vi "Read Boolean.vi"(8 "error in":errorcluster, 9 "RegisterOffset":u32, 10 "register name":string, 11 "session in":u32) -> (0 "error out":errorcluster, 2 "value out":bool, 3 "session out":u32)   [LabVIEW 2020, in "FPGA Register IO.lvlib"]
uses:
  FPGA Register IO.lvlib
  NiFpga.dll
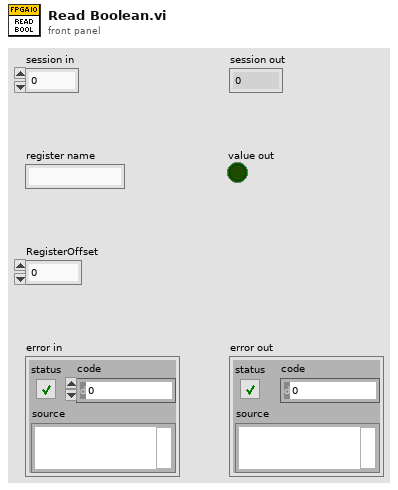
[diagram p1: front panel]
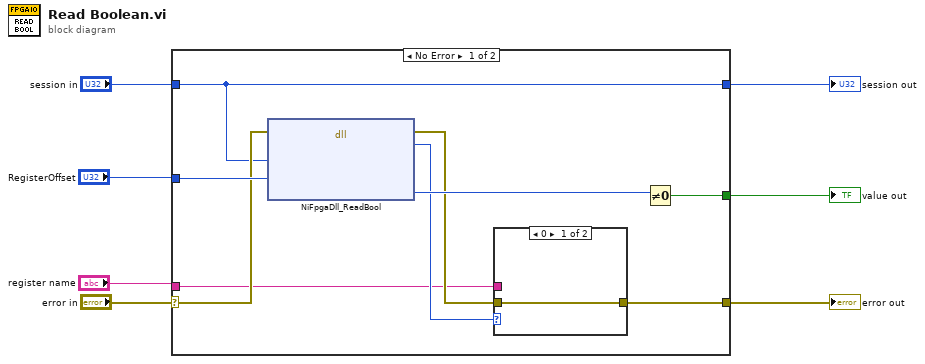
[diagram p0: block diagram]
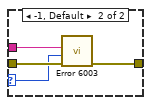
[diagram p2: hidden frame]
diagram:
  n1 = case shown="No Error" "error in" {
    selector: "error in" -> [w15 w23]
    tunnel: "session in" -> [w14 w22]
    tunnel: [w9 w23] -> w7
    tunnel: [w13 _] -> w5
    tunnel: "RegisterOffset" -> [w16 _]
    tunnel: [w14 w22] -> w6
    tunnel: "register name" -> [w8 _]
    frame No Error {
      n2 = dll-call lib="NiFpga.*" fn="NiFpgaDll_ReadBool"(error in=w15, "session"=w14, "offset"=w16) -> (error out=w10:errorcluster, "status"=w11:i32, "value"=w12:u8)  [unwired: 5 in, 1 out]
      n3 = case shown="0" w11 {
        selector: w11 -> [_ w18]
        tunnel: w10 -> [w17 w21]
        tunnel: [w17 w20] -> w9
        tunnel: w8 -> [_ w19]
        frame 0 {
        }
        frame -1, Default {
          n4 = call "Error 6003.vi"("error in (no error)"=w21, "rio status code"=w18, "register name"=w19) -> ("error out"=w20:errorcluster)  [unwired: 8 in]
        }
      }
      n5 = Not Equal To 0?(x=w12) -> (x != 0?=w13:bool)
    }
    frame Error {
    }
  }
  "error out" <- w7
  "session out" <- w6
  "value out" <- w5
